vi "csb hdlc decode.vi"(0 "state":u8[](array[numeric]), 1 "state_size":i32, 2 "in":u8[](array[numeric]), 3 "in_len":i32, 4 "out":u8[](array[numeric]), 5 "out_cap":i32, 6 "lens":i32[](array[numeric]), 7 "error in (no error)":errorcluster, 8 "lens_cap":i32) -> (20 "state out":u8[](array[numeric]), 21 "n_payloads":i32, 22 "crc_errors":u32, 23 "function return":i32, 24 "out out":u8[](array[numeric]), 26 "lens out":i32[](array[numeric]), 27 "error out":errorcluster)   [LabVIEW 2021, in "CANsub_Codec.lvlib"]
doc: "int32_t csb_hdlc_decode(uint8_t *state, int32_t state_size,\n const uint8_t *in, int32_t in_len,\n uint8_t *out, int32_t out_cap,\n int32_t *lens, int32_t lens_cap,\n int32_t *n_payloads, uint32_t *crc_errors);"
uses:
  CANsub_Codec.lvlib
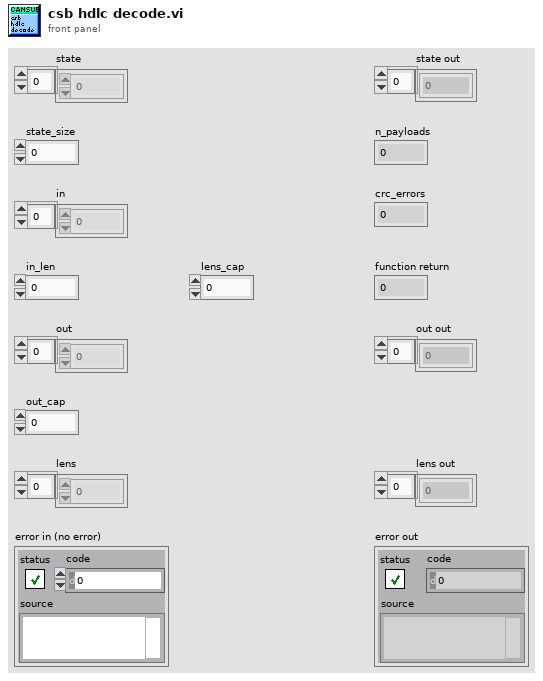
[diagram p1: front panel]
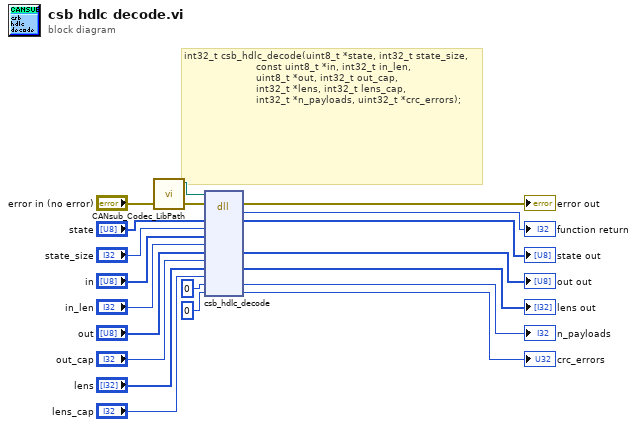
[diagram p0: block diagram]
diagram:
  # "int32_t csb_hdlc_decode(uint8_t *state, int32_t state_size,\n                        const uint8_t *in, int32_t in_len,\n                        uint8_t *out, int32_t out_cap,\n                        int32_t *lens, int32_t lens_cap,\n                        int32_t *n_payloads, uint32_t *crc_errors);"
  n1 = call "CANsub_Codec_LibPath.vi"() -> ("Path"=w1:path)  [unwired: 11 in]
  n2 = dll-call lib="libcansub_codec.*" fn="csb_hdlc_decode"(path in=w1, error in="error in (no error)", "state"="state", "state_size"="state_size", "in"="in", "in_len"="in_len", "out"="out", "out_cap"="out_cap", "lens"="lens", "lens_cap"="lens_cap", "n_payloads"=0, "crc_errors"=u32 0) -> (error out=→"error out":errorcluster, "return type"=→"function return":i32, "state"=→"state out":u8[], "out"=→"out out":u8[], "lens"=→"lens out":i32[], "n_payloads"=→"n_payloads":i32, "crc_errors"=→"crc_errors":u32)  [unwired: 6 in, 1 out]
